vi "identify classes in memory.vi"(8 "error in":errorcluster, 10 "class cache data in":T1, 11 "Path":path) -> (0 "error out":errorcluster, 2 "class cache data out":T1)   [LabVIEW 2013, in "PL_class cache.lvlib"]
uses:
  PL_class cache.lvlib
  cached class information.ctl
  target class metadata.ctl
  class metadata.ctl
  <vilib>/NI/Tag Bus Module Framework/root configuration/Target Types.ctl
  Configuration Editor/Classes/Targets/Targets.lvclass
  Configuration Editor/Classes/Engine Parent/Engine Parent Editor Node.lvclass
  <vilib>/NI/Tag Bus Module Framework/root configuration/TBM configuration.lvclass
  <vilib>/NI/Configuration Framework/serializable configuration/NISE_CEF_serializable configuration.lvclass
  Configuration Editor/Classes/Module editor node/module editor node.lvclass
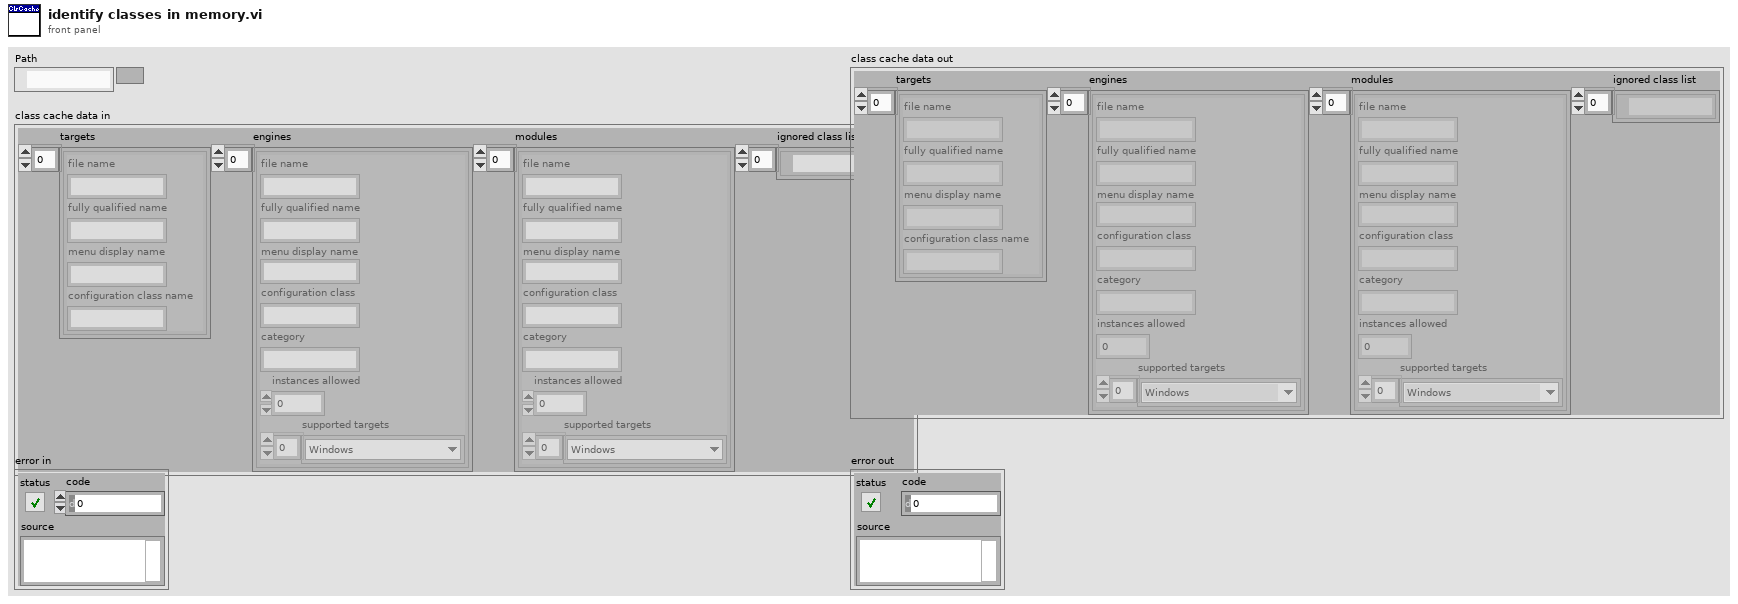
[diagram p1: front panel]
types:
  T1 = typedef "PL_class cache.lvlib/cached class information.ctl" = cluster{"targets":T2[], "engines":T3[], "modules":T3[], "ignored class list":path[]}
  T2 = typedef "PL_class cache.lvlib/target class metadata.ctl" = cluster{"file name":string, "fully qualified name":string, "menu display name":string, "configuration class name":string}
  T3 = typedef "PL_class cache.lvlib/class metadata.ctl" = cluster{"file name":string, "fully qualified name":string, "menu display name":string, "configuration class":string, "category":string, "instances allowed":i32, "supported targets":T4[]}
  T4 = typedef "TBM configuration.lvclass/Target Types.ctl" = enum16{"Windows", "Mac", "Linux", "Linux RT ARM", "VxWorks", "Pharlap", "Other", "Linux RT x64"}
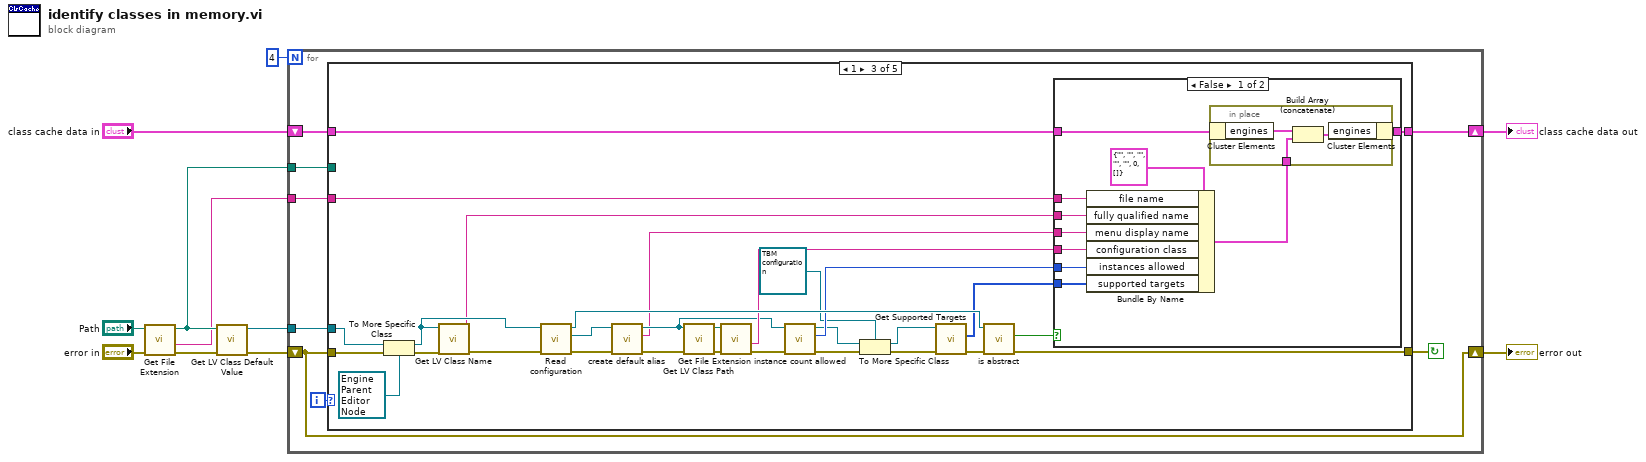
[diagram p0: block diagram]
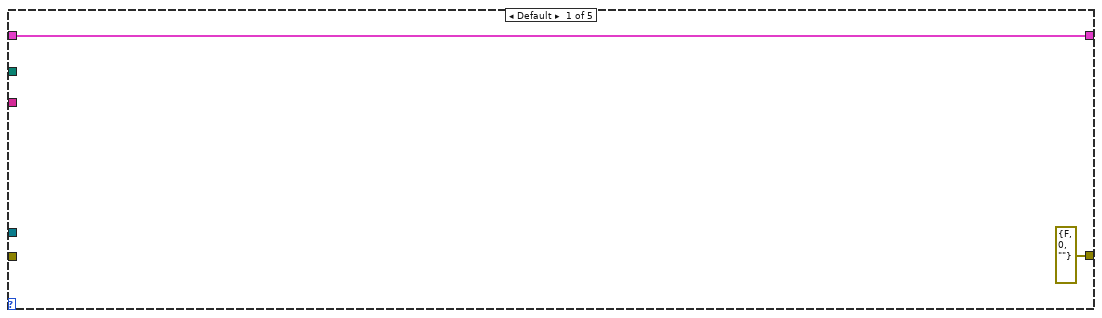
[diagram p2: hidden frame]
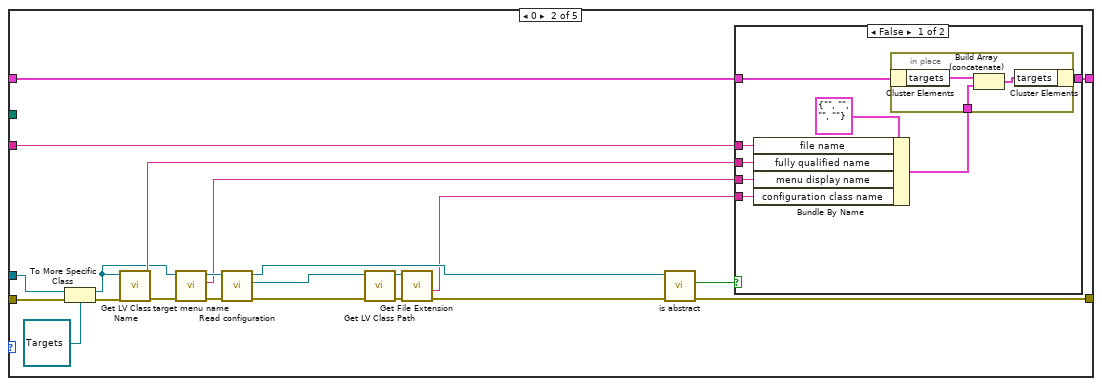
[diagram p3: hidden frame]
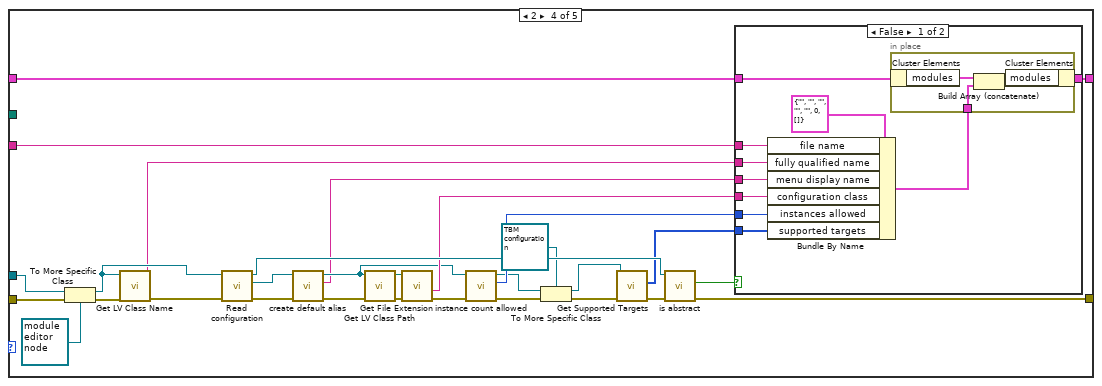
[diagram p6: hidden frame]
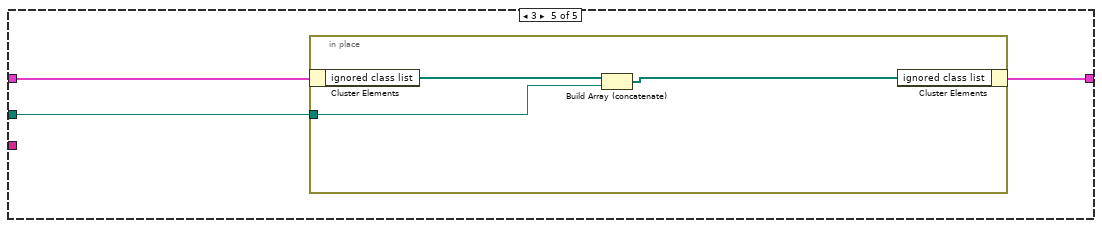
[diagram p8: hidden frame]
diagram:
  n1 = call <vilib>:"Get File Extension.vi"("error in (no error)"="error in", "file"="Path") -> ("error out"=w10:errorcluster, "filename without extension"=w1:string, "dup file"=w2:path)  [unwired: 6 in, 1 out]
  n2 = call <vilib>:"Get LV Class Default Value.vi"("error in (no error)"=w10, "class path"=w2) -> ("error out"=w8:errorcluster, "object"=w7:refnum<class>)  [unwired: 8 in]
  n3 = for {
    N: 4 -> [_]
    shift-right: [w16] -> w3
    shift-left: w8 -> [w16]
    tunnel: w7 -> [w15]
    tunnel: w1 -> [w13]
    shift-right: [w17] -> w4
    shift-left: "class cache data in" -> [w18]
    tunnel: w2 -> [w12]
    i -> [w19]
    stop <- w14 continue-if-true
    n4 = case shown="1" w19 {
      tunnel: w18 -> [w21 w33 w75 w119 w146]
      tunnel: [w21 w32 w74 w118 w145] -> w17
      tunnel: w16 -> [_ w43 w85 w129 _]
      tunnel: w15 -> [_ w42 w84 w128 _]
      tunnel: [errorcluster {"status"=FALSE, "code"=0, "source"=""} ("error out") w34 w76 w120 _] -> w14
      tunnel: w13 -> [_ w30 w72 w116 _]
      tunnel: w12 -> [_ _ _ _ w144]
      frame Default {
      }
      frame 0 {
        n5 = To More Specific Class(target class=refnum<class "Targets.lvclass"> refnum ("Targets"), reference=w42, error in=w43) -> (specific class reference=w25:refnum<class "Targets.lvclass">, error out=w40:errorcluster)
        n6 = call <vilib>:"Get LV Class Name.vi"("error in (no error)"=w40, "object"=w25) -> ("error out"=w24:errorcluster, "class name"=w31:string)  [unwired: 8 in]
        n7 = call-dynamic "target menu name.vi"("error in"=w24, "Targets in"=w25) -> ("error out"=w23:errorcluster, "menu name"=w22:string, "Targets out"=w26:refnum<class "Targets.lvclass">)  [unwired: 7 in]
        n8 = call-dynamic "Read configuration.vi"("error in"=w23, "NISE_CEF_serializable node in"=w26) -> ("error out"=w36:errorcluster, "configuration"=w27:refnum<class "NISE_CEF_serializable configuration.lvclass">, "NISE_CEF_serializable node out"=w38:refnum<class "Targets.lvclass">)  [unwired: 7 in]
        n9 = call <vilib>:"Get LV Class Path.vi"("error in (no error)"=w36, "object"=w27) -> ("error out"=w37:errorcluster, "class path"=w35:path)  [unwired: 8 in]
        n10 = call <vilib>:"Get File Extension.vi"("error in (no error)"=w37, "file"=w35) -> ("error out"=w39:errorcluster, "filename without extension"=w29:string)  [unwired: 6 in, 2 out]
        n11 = call-dynamic "is abstract.vi"("error in"=w39, "Targets in"=w38) -> ("error out"=w34:errorcluster, "abstract"=w28:bool)  [unwired: 7 in, 1 out]
        n12 = case shown="False" w28 {
          tunnel: w33 -> [w49 w55]
          tunnel: [w48 w55] -> w32
          tunnel: w31 -> [w47 _]
          tunnel: w30 -> [w46 _]
          tunnel: w22 -> [w45 _]
          tunnel: w29 -> [w44 _]
          frame False {
            n13 = Bundle By Name(cluster=T2 {"file name"="", "fully qualified name"="", "menu display name"="", "configuration class name"=""} ("class metadata"), "file name"=w46, "fully qualified name"=w47, "menu display name"=w45, "configuration class name"=w44) -> (w50:T2)
            n14 = in-place {
              in-place-border: w50 -> [w52]
              n15 = in-place-cluster #1(w49) -> ("targets"=w54:T2[])
              n16 = Build Array (concatenate)(w54, w52) -> (w53:T2[])
              n17 = in-place-cluster #1("targets"=w53) -> (w48:T1)
            }
          }
          frame True {
          }
        }
      }
      frame 1 {
        n18 = To More Specific Class(target class=refnum<class "Engine Parent Editor Node.lvclass"> refnum ("Engine Parent.lvclass"), reference=w84, error in=w85) -> (specific class reference=w77:refnum<class "Engine Parent Editor Node.lvclass">, error out=w83:errorcluster)
        n19 = call <vilib>:"Get LV Class Name.vi"("error in (no error)"=w83, "object"=w77) -> ("error out"=w56:errorcluster, "class name"=w73:string)  [unwired: 8 in]
        n20 = call-dynamic "Read configuration.vi"("error in"=w56, "NISE_CEF_serializable node in"=w77) -> ("error out"=w79:errorcluster, "configuration"=w59:refnum<class "NISE_CEF_serializable configuration.lvclass">, "NISE_CEF_serializable node out"=w81:refnum<class "Engine Parent Editor Node.lvclass">)  [unwired: 7 in]
        n21 = call-dynamic "create default alias.vi"("error in"=w79, "configuration in"=w59) -> ("error out"=w60:errorcluster, "default alias"=w57:string, "configuration out"=w58:refnum<class "NISE_CEF_serializable configuration.lvclass">)  [unwired: 7 in]
        n22 = call <vilib>:"Get LV Class Path.vi"("error in (no error)"=w60, "object"=w58) -> ("error out"=w80:errorcluster, "class path"=w78:path)  [unwired: 8 in]
        n23 = call <vilib>:"Get File Extension.vi"("error in (no error)"=w80, "file"=w78) -> ("error out"=w82:errorcluster, "filename without extension"=w71:string)  [unwired: 6 in, 2 out]
        n24 = call-dynamic "instance count allowed.vi"("error in"=w82, "configuration in"=w58) -> ("error out"=w68:errorcluster, "instances allowed"=w66:i32, "configuration out"=w61:refnum<class "NISE_CEF_serializable configuration.lvclass">)  [unwired: 7 in]
        n25 = To More Specific Class(target class=refnum<class "TBM configuration.lvclass"> refnum ("configuration in"), reference=w61, error in=w68) -> (specific class reference=w63:refnum<class "TBM configuration.lvclass">, error out=w64:errorcluster)
        n26 = call-dynamic "Get Supported Targets.vi"("error in"=w64, "configuration in"=w63) -> ("error out"=w67:errorcluster, "supported targets"=w65:T4[])  [unwired: 7 in, 1 out]
        n27 = call-dynamic "is abstract.vi"("error in"=w67, "Engine Parent Editor Node in"=w81) -> ("error out"=w76:errorcluster, "abstract"=w70:bool)  [unwired: 7 in, 1 out]
        n28 = case shown="False" w70 {
          tunnel: w75 -> [w94 w99]
          tunnel: [w93 w99] -> w74
          tunnel: w73 -> [w92 _]
          tunnel: w72 -> [w91 _]
          tunnel: w57 -> [w90 _]
          tunnel: w71 -> [w89 _]
          tunnel: w66 -> [w87 _]
          tunnel: w65 -> [w86 _]
          frame False {
            n29 = Bundle By Name(cluster=T3 {"file name"="", "fully qualified name"="", "menu display name"="", "configuration class"="", "category"="", "instances allowed"=0, "supported targets"=[]} ("class metadata"), "file name"=w91, "fully qualified name"=w92, "menu display name"=w90, "configuration class"=w89, "instances allowed"=w87, "supported targets"=w86) -> (w95:T3)
            n30 = in-place {
              in-place-border: w95 -> [w96]
              n31 = in-place-cluster #2(w94) -> ("engines"=w98:T3[])
              n32 = Build Array (concatenate)(w98, w96) -> (w97:T3[])
              n33 = in-place-cluster #2("engines"=w97) -> (w93:T1)
            }
          }
          frame True {
          }
        }
      }
      frame 2 {
        n34 = To More Specific Class(target class=refnum<class "module editor node.lvclass"> refnum ("Component Parent.lvclass"), reference=w128, error in=w129) -> (specific class reference=w121:refnum<class "module editor node.lvclass">, error out=w127:errorcluster)
        n35 = call <vilib>:"Get LV Class Name.vi"("error in (no error)"=w127, "object"=w121) -> ("error out"=w100:errorcluster, "class name"=w117:string)  [unwired: 8 in]
        n36 = call-dynamic "Read configuration.vi"("error in"=w100, "NISE_CEF_serializable node in"=w121) -> ("error out"=w123:errorcluster, "configuration"=w103:refnum<class "NISE_CEF_serializable configuration.lvclass">, "NISE_CEF_serializable node out"=w125:refnum<class "module editor node.lvclass">)  [unwired: 7 in]
        n37 = call-dynamic "create default alias.vi"("error in"=w123, "configuration in"=w103) -> ("error out"=w104:errorcluster, "default alias"=w101:string, "configuration out"=w102:refnum<class "NISE_CEF_serializable configuration.lvclass">)  [unwired: 7 in]
        n38 = call <vilib>:"Get LV Class Path.vi"("error in (no error)"=w104, "object"=w102) -> ("error out"=w124:errorcluster, "class path"=w122:path)  [unwired: 8 in]
        n39 = call <vilib>:"Get File Extension.vi"("error in (no error)"=w124, "file"=w122) -> ("error out"=w126:errorcluster, "filename without extension"=w115:string)  [unwired: 6 in, 2 out]
        n40 = call-dynamic "instance count allowed.vi"("error in"=w126, "configuration in"=w102) -> ("error out"=w113:errorcluster, "instances allowed"=w111:i32, "configuration out"=w107:refnum<class "NISE_CEF_serializable configuration.lvclass">)  [unwired: 7 in]
        n41 = To More Specific Class(target class=refnum<class "TBM configuration.lvclass"> refnum ("configuration in"), reference=w107, error in=w113) -> (specific class reference=w105:refnum<class "TBM configuration.lvclass">, error out=w108:errorcluster)
        n42 = call-dynamic "Get Supported Targets.vi"("error in"=w108, "configuration in"=w105) -> ("error out"=w112:errorcluster, "supported targets"=w110:T4[])  [unwired: 7 in, 1 out]
        n43 = call-dynamic "is abstract.vi"("error in"=w112, "module editor node in"=w125) -> ("error out"=w120:errorcluster, "abstract"=w114:bool)  [unwired: 7 in, 1 out]
        n44 = case shown="False" w114 {
          tunnel: w119 -> [w138 w143]
          tunnel: [w137 w143] -> w118
          tunnel: w117 -> [w136 _]
          tunnel: w116 -> [w135 _]
          tunnel: w101 -> [w134 _]
          tunnel: w115 -> [w133 _]
          tunnel: w111 -> [w131 _]
          tunnel: w110 -> [w130 _]
          frame False {
            n45 = Bundle By Name(cluster=T3 {"file name"="", "fully qualified name"="", "menu display name"="", "configuration class"="", "category"="", "instances allowed"=0, "supported targets"=[]} ("class metadata"), "file name"=w135, "fully qualified name"=w136, "menu display name"=w134, "configuration class"=w133, "instances allowed"=w131, "supported targets"=w130) -> (w139:T3)
            n46 = in-place {
              in-place-border: w139 -> [w140]
              n47 = in-place-cluster #3(w138) -> ("modules"=w142:T3[])
              n48 = Build Array (concatenate)(w142, w140) -> (w141:T3[])
              n49 = in-place-cluster #3("modules"=w141) -> (w137:T1)
            }
          }
          frame True {
          }
        }
      }
      frame 3 {
        n50 = in-place {
          in-place-border: w144 -> [w147]
          n51 = in-place-cluster #4(w146) -> ("ignored class list"=w149:path[])
          n52 = Build Array (concatenate)(w149, w147) -> (w148:path[])
          n53 = in-place-cluster #4("ignored class list"=w148) -> (w145:T1)
        }
      }
    }
  }
  "class cache data out" <- w4
  "error out" <- w3
